vi "Stop Core.vi"(10 "final error code":i32, 11 "Nested in":refnum<class "DIO_Panel.lvclass">) -> (3 "Nested out":refnum<class "DIO_Panel.lvclass">)   [LabVIEW 2021, in "Simulator-Channel.lvlib" / "DIO_Panel.lvlib" / "DIO_Panel.lvclass"]
doc: "(<B>Filename</B>: Actor Framework.lvlib:Actor.lvclass:Stop Core.vi)\n\nDefines what the actor does before it stops. Use the <B>final error code</B> input to determine whether the actor shut down in response to an error.\n\nBy default, this method does nothing. A descendant class may override it to define behavior, such as shutting down any processes the actor initiated in its override of the Actor Core method."
uses:
  DIO_Panel.lvclass
  <vilib>/event_ctls.llb/usereventprio.ctl
  <vilib>/ActorFramework/Message Enqueuer/Message Enqueuer.lvclass
  DIO_Panel.lvclass/DIO_Panel.ctl
  Channels/DIO-Channel/Private/G_Variables.vi
  <vilib>/ActorFramework/Actor/Actor.lvclass
  Channels/DIO-Channel/Simulator-Channel.lvlib
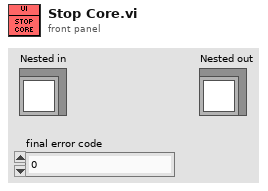
[diagram p1: front panel]
types:
  T1 = typedef "usereventprio.ctl" = enum32{"high priority", "normal priority"}
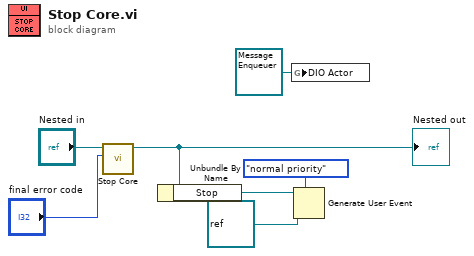
[diagram p0: block diagram]
diagram:
  n1 = call-parent "Stop Core.vi"("final error code"="final error code", "Actor in"="Nested in") -> ("Actor out"=w5:refnum<class "DIO_Panel.lvclass">)  [unwired: 9 in]
  "Nested out" <- w5
  n2 = Unbundle By Name(w5) -> ("Stop"=w4:refnum<user-event>)
  n3 = global write "G_Variables.vi" "DIO Actor"(refnum<class "Message Enqueuer.lvclass"> refnum ("DIO Actor")) -> ()
  n4 = Generate User Event(priority (normal)=usereventprio."normal priority", user event=w4, event data cluster=refnum<class> refnum ("event data")) -> ()  [unwired: 1 in, 2 out]
